vi "H12_Station_Name.vi"() -> ()   [LabVIEW 2026]
doc: "Use this template to build a VI to use as a subVI."
uses:
  kernel32.dll
panel:
  out "error out":errorcluster
  out "name length":u32
  out "station name":string
  out "call 2 ok (1 = success)":i32
  out "size needed":u32
  out "call 1 ok (0 = buffer too small)":i32
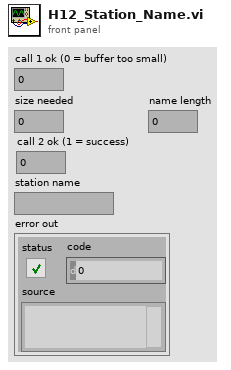
[diagram p1: front panel]
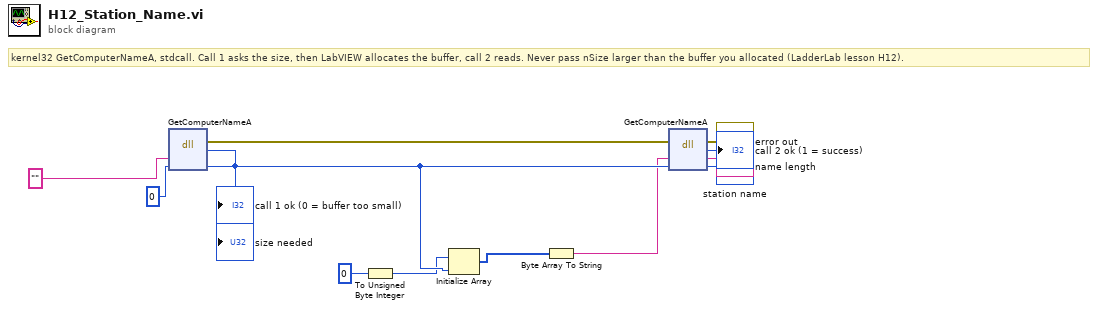
[diagram p0: block diagram]
diagram:
  # "kernel32 GetComputerNameA, stdcall. Call 1 asks the size, then LabVIEW allocates the buffer, call 2 reads. Never pass nSize larger than the buffer you allocated (LadderLab lesson H12)."
  n1 = dll-call lib="kernel32.dll" fn="GetComputerNameA"("lpBuffer"="", "nSize"=u32 0) -> (error out=w6:errorcluster, →"call 1 ok (0 = buffer too small)":i32, "nSize"=w10:u32)  [unwired: 4 in, 1 out]
  "size needed" <- w10
  n2 = To Unsigned Byte Integer(number=u8 0) -> (unsigned 8bit integer=w9:u8)
  n3 = Initialize Array(w9, w10) -> (w8:u8[])
  n4 = Byte Array To String(unsigned byte array=w8) -> (string=w7:string)
  n5 = dll-call lib="kernel32.dll" fn="GetComputerNameA"(error in=w6, "lpBuffer"=w7, "nSize"=w10) -> (error out=→"error out":errorcluster, →"call 2 ok (1 = success)":i32, "lpBuffer"=→"station name":string, "nSize"=→"name length":u32)  [unwired: 2 in, 1 out]
